vi "Set ROI v2.vi"(8 "error in (no error)":errorcluster, 10 "ROI":T1, 11 "HamamatsuFluor in":refnum<class "HamamatsuFluor.lvclass">) -> (0 "error out":errorcluster, 3 "HamamatsuFluor out":refnum<class "HamamatsuFluor.lvclass">)   [LabVIEW 2020, in "DAQ Timed SPIM.lvlib" / "HamamatsuFluor_v2.lvlib" / "HamamatsuFluor.lvclass"]
uses:
  HamamatsuFluor.lvclass
  HamamatsuFluor.lvclass/HamamatsuFluor.ctl
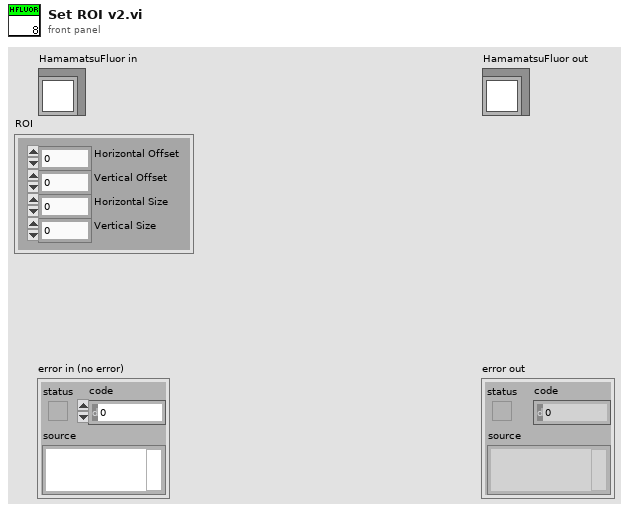
[diagram p1: front panel]
types:
  T1 = cluster{"Horizontal Offset":i32, "Vertical Offset":i32, "Horizontal Size":i32, "Vertical Size":i32}
  T2 = typedef "LVMinMaxIncTypeDef.ctl" = cluster{"Minimum":dbl, "Maximum":dbl, "Increment":dbl}
  T3 = cluster{"H Offset":cluster{"Value":i32, "Limits":T2}, "V Offset":cluster{"Value":i32, "Limits":T2}, "H Size":cluster{"Value":i32, "Limits":T2}, "V Size":cluster{"Value":i32, "Limits":T2}}
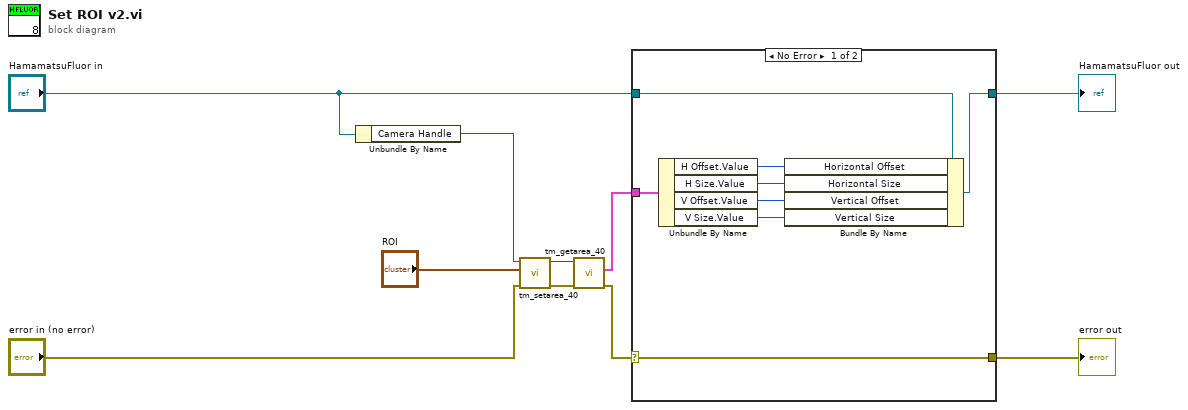
[diagram p0: block diagram]
diagram:
  n1 = Unbundle By Name("HamamatsuFluor in") -> ("Camera Handle"=w9:u32)
  n2 = call <userlib>:"tm_setarea_40.vi"("error in (no error)"="error in (no error)", "Sub Region"="ROI", "Handle in"=w9) -> ("error out"=w8:errorcluster, "Handle out"=w7:u32)  [unwired: 7 in]
  n3 = call <userlib>:"tm_getarea_40.vi"("error in (no error)"=w8, "Handle in"=w7) -> ("error out"=w5:errorcluster, "Sub Region"=w6:T3)  [unwired: 7 in, 1 out]
  n4 = case shown="No Error" w5 {
    selector: w5 -> [w17 w20]
    tunnel: w6 -> [w18 _]
    tunnel: [w17 w20] -> w4
    tunnel: "HamamatsuFluor in" -> [w16 w19]
    tunnel: [w11 w19] -> w2
    frame No Error {
      n5 = Unbundle By Name(w18) -> ("H Offset.Value"=w15:i32, "H Size.Value"=w14:i32, "V Offset.Value"=w13:i32, "V Size.Value"=w12:i32)
      n6 = Bundle By Name(cluster=w16, "Horizontal Offset"=w15, "Horizontal Size"=w14, "Vertical Offset"=w13, "Vertical Size"=w12) -> (w11:refnum<class "HamamatsuFluor.lvclass">)
    }
    frame Error {
    }
  }
  "error out" <- w4
  "HamamatsuFluor out" <- w2
